vi "Increment.vi"(6 "Labels":map{string, string}(c390), 8 "error in (no error)":errorcluster, 10 "Step":dbl=1.0, 11 "Counter Ref":refnum<data-value>) -> (0 "error out":errorcluster, 3 "Counter Ref out":refnum<data-value>)   [LabVIEW 2020, in "Metrics.lvlib" / "Counter.lvclass"]
doc: "Increments the value of the counter. By default, the increment value is 1."
uses:
  Counter.lvclass
  C:/Github-locals/PromVIEW/src/metrics/metric/Metric.lvclass
  sample/Edit Action.ctl
  metric/Metric.lvclass
  sample/Sample.lvclass
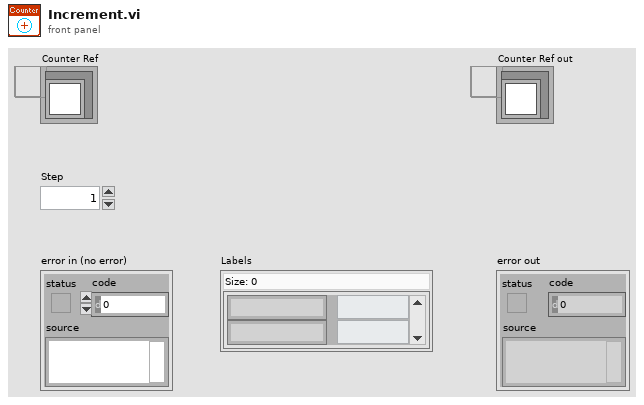
[diagram p1: front panel]
types:
  T1 = typedef "Metrics.lvlib/Sample.lvclass/Edit Action.ctl" = enum16{"Set", "Increment"}
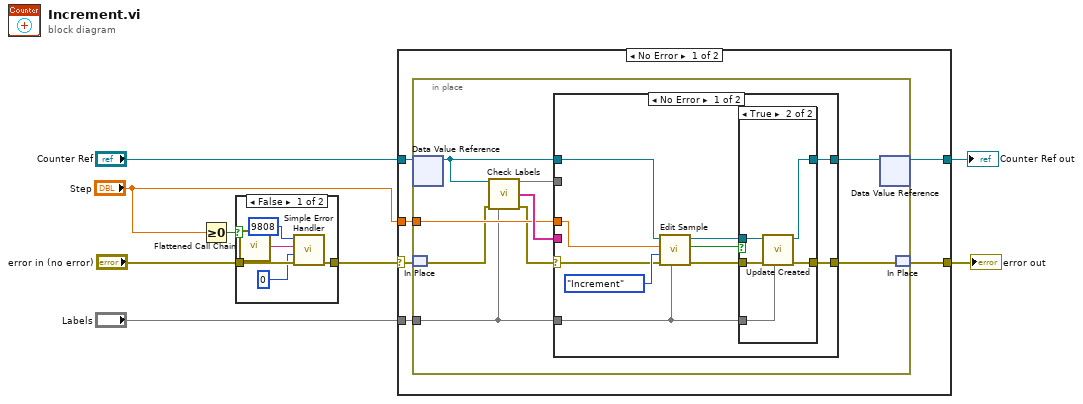
[diagram p0: block diagram]
diagram:
  n1 = Greater Or Equal To 0?(x="Step") -> (x >= 0?=w7:bool)
  n2 = case shown="False" w7 {
    tunnel: "error in (no error)" -> [w12 w14]
    tunnel: [w11 w14] -> w5
    frame False {
      n3 = call "Flattened Call Chain.vi"() -> ("Flattened Call Chain"=w10:string)  [unwired: 5 in]
      n4 = call <vilib>:"Simple Error Handler.vi"("error code (no error:0)"=9808, "error source (\" \")"=w10, "type of dialog (OK msg:1)"=0 ("error code (no error:0)"), "error in (no error)"=w12) -> ("error out"=w11:errorcluster)  [unwired: 1 in, 4 out]
    }
    frame True {
    }
  }
  n5 = case shown="No Error" w5 {
    selector: w5 -> [w19 w49]
    tunnel: "Counter Ref" -> [w20 w50]
    tunnel: "Labels" -> [w18 _]
    tunnel: "Step" -> [w17 _]
    tunnel: [w16 w49] -> w2
    tunnel: [w15 w50] -> w1
    frame No Error {
      n6 = in-place {
        in-place-border: w18 -> [w25]
        in-place-border: w17 -> [w26]
        n7 = in-place-dvr #1(w20) -> (w29:refnum<class "Counter.lvclass">)  [unwired: 1 out]
        n8 = in-place-match #2(w19) -> (w22:errorcluster)
        n9 = call-dynamic "Check Labels.vi"("Metric in"=w29, "error in (no error)"=w22, "Labels"=w25) -> ("Samples"=w27:map{string, refnum<class "Sample.lvclass">}, "Label Values"=w28:string[], "error out"=w21:errorcluster)  [unwired: 9 in, 1 out]
        n10 = case shown="No Error" w21 {
          selector: w21 -> [w34 w47]
          tunnel: w28 -> [_ _]
          tunnel: w27 -> [_ _]
          tunnel: w26 -> [w36 _]
          tunnel: w25 -> [w30 _]
          tunnel: [w39 w47] -> w24
          tunnel: w29 -> [w37 w48]
          tunnel: [w38 w48] -> w23
          frame No Error {
            n11 = call "Edit Sample.vi"("Labels"=w30, "error in (no error)"=w34, "Action"=Edit_Action."Increment", "Step"=w36, "Metric in"=w37) -> ("error out"=w31:errorcluster, "New Sample?"=w32:bool, "Metric out"=w33:refnum<class "Counter.lvclass">)  [unwired: 4 in]
            n12 = case shown="True" w32 {
              tunnel: w31 -> [w41 w46]
              tunnel: [w41 w45] -> w39
              tunnel: w30 -> [_ w44]
              tunnel: w33 -> [w40 w43]
              tunnel: [w40 w42] -> w38
              frame False {
              }
              frame True {
                n13 = call "Update Created.vi"("Labels"=w44, "error in (no error)"=w46, "Counter in"=w43) -> ("error out"=w45:errorcluster, "Counter out"=w42:refnum<class "Counter.lvclass">)  [unwired: 7 in]
              }
            }
          }
          frame Error {
          }
        }
        n14 = in-place-dvr #1(w23) -> (w15:refnum<data-value>)  [unwired: 1 out]
        n15 = in-place-match #2(w24) -> (w16:errorcluster)
      }
    }
    frame Error {
    }
  }
  "error out" <- w2
  "Counter Ref out" <- w1
